vi "Initialization.vi"(8 "error in (no error)":errorcluster, 9 "UI Refs":T1, 10 "user event":T2, 11 "4way Lap in":refnum<class "No Load Drift.lvclass">) -> (0 "error out":errorcluster, 3 "4way Lap out":refnum<class "No Load Drift.lvclass">)   [LabVIEW 2025, in "Flow Grind.lvlib" / "No Load Drift.lvclass"]
uses:
  No Load Drift.lvclass
  Users/Public/Documents/Sandia National Labs/TSS Plugin/CEF.lvlibp/Node/UserEventRef.ctl
  Users/Public/Documents/Sandia National Labs/TSS Plugin/Tests/XY Plotter.lvlibp/XY  Plotter/XY Plotter.lvclass
  Users/Public/Documents/Sandia National Labs/TSS Plugin/CEF.lvlibp/Node/CEF_Node.lvclass
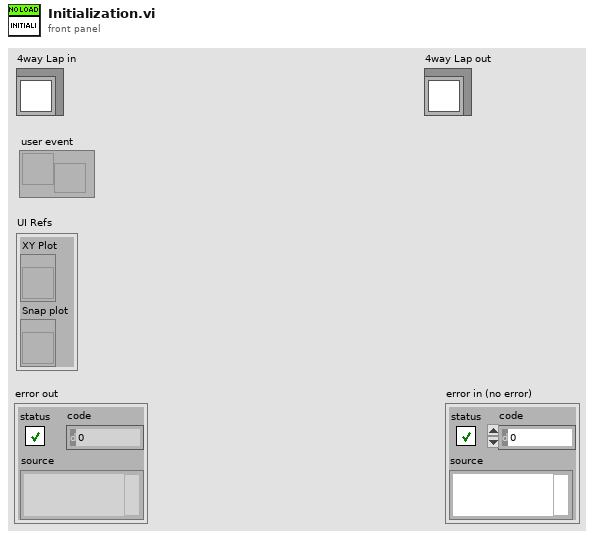
[diagram p1: front panel]
types:
  T1 = cluster{"XY Plot":refnum<vi>, "Snap plot":refnum<vi>}
  T2 = typedef "CEF.lvlibp/CEF_Node.lvclass/UserEventRef.ctl" = refnum<user-event>
  T3 = cluster{"Name":string, "Color":u32, "Style":u8, "Point Style":u8, "Name Visible":bool, "Allow Drag":bool, "Annotation Mode":u32, "Plot":i32, "Index":i32, "Position":cluster{"X":dbl, "Y":dbl}, "X Scale":u32, "Y Scale":u32, "Show Arrow":bool, "Lock Name":bool, "Plot Area":i32, "Label Offset":cluster{"X":dbl, "Y":dbl}}
  T4 = cluster{"Name":string, "Color":u32, "Style":u8, "Point Style":u8, "Name Visible":bool, "Allow Drag":bool, "Annotation Mode":u32, "Plot":i32, "Index":i32, "Position":cluster{"X":dbl, "Y":dbl}, "X Scale":u32, "Y Scale":u32, "Show Arrow":bool, "Lock Name":bool, "Plot Area":i32, "Label Offset":cluster{"X":dbl, "Y":dbl}}[]
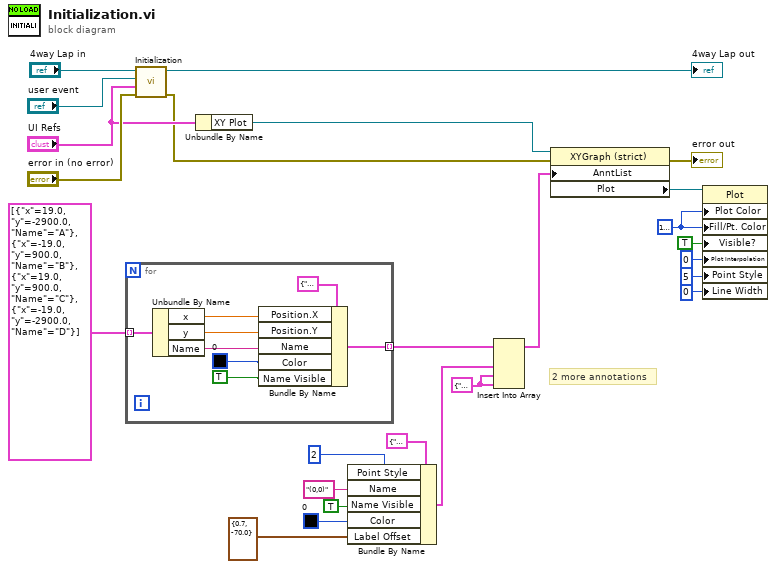
[diagram p0: block diagram]
diagram:
  w8 = T3 {"Name"="", "Color"=0, "Style"=0, "Point Style"=0, "Name Visible"=FALSE, "Allow Drag"=FALSE, "Annotation Mode"=0, "Plot"=0, "Index"=0, "Position"={"X"=0.0, "Y"=0.0}, "X Scale"=0, "Y Scale"=0, "Show Arrow"=FALSE, "Lock Name"=FALSE, "Plot Area"=0, "Label Offset"={"X"=0.0, "Y"=0.0}} ("new element/subarray")
  w17 = u32 16777224 ("Plot Color")
  # "2 more annotations"
  n1 = for {
    tunnel: cluster{"x":dbl, "y":dbl, "Name":string}[] [{"x"=19.0, "y"=-2900.0, "Name"="A"}, {"x"=-19.0, "y"=900.0, "Name"="B"}, {"x"=19.0, "y"=900.0, "Name"="C"}, {"x"=-19.0, "y"=-2900.0, "Name"="D"}] -> [w29] mode=indexing
    tunnel: [w30] -> w12 mode=indexing
    n2 = Unbundle By Name(w29) -> ("x"=w27:dbl, "y"=w26:dbl, "Name"=w28:string)
    n3 = Bundle By Name(cluster=T3 {"Name"="", "Color"=0, "Style"=0, "Point Style"=0, "Name Visible"=FALSE, "Allow Drag"=FALSE, "Annotation Mode"=0, "Plot"=0, "Index"=0, "Position"={"X"=0.0, "Y"=0.0}, "X Scale"=0, "Y Scale"=0, "Show Arrow"=FALSE, "Lock Name"=FALSE, "Plot Area"=0, "Label Offset"={"X"=0.0, "Y"=0.0}}, "Position.X"=w27, "Position.Y"=w26, "Name"=w28, "Color"=u32 0, "Name Visible"=TRUE) -> (w30:T3)
  }
  n4 = call-parent "Initialization.vi"("error in"="error in (no error)", "UI Refs"="UI Refs", "user event"="user event", "XY Plotter"="4way Lap in") -> ("error out"=w14:errorcluster, "XY Plotter out"=→"4way Lap out":refnum<class "No Load Drift.lvclass">)  [unwired: 6 in]
  n5 = Unbundle By Name("UI Refs") -> ("XY Plot"=w10:refnum<vi>)
  n6 = Bundle By Name(cluster=T3 {"Name"="", "Color"=0, "Style"=0, "Point Style"=0, "Name Visible"=FALSE, "Allow Drag"=FALSE, "Annotation Mode"=0, "Plot"=0, "Index"=0, "Position"={"X"=0.0, "Y"=0.0}, "X Scale"=0, "Y Scale"=0, "Show Arrow"=FALSE, "Lock Name"=FALSE, "Plot Area"=0, "Label Offset"={"X"=0.0, "Y"=0.0}} ("new element/subarray"), "Point Style"=u8 2, "Name"="(0,0)", "Name Visible"=TRUE, "Color"=u32 0, "Label Offset"=cluster{"X":dbl, "Y":dbl} {"X"=0.7, "Y"=-70.0}) -> (w1:T3)
  n7 = Insert Into Array(array=w12, new element #1=w1, new element #2=w8, new element #3=w8) -> (w11:T4)  [unwired: 1 in]
  n8 = property class="XYGraph (strict)"(reference=w10, error in=w14, "AnntList"=w11) -> (error out=→"error out":errorcluster, "Plot"=w9:refnum<vi>)  [unwired: 1 out]
  n9 = property class="Plot"(reference=w9, "Plot Color"=w17, "Fill/Pt. Color"=w17, "Visible?"=TRUE ("Visible"), "Plot Interpolation"=u8 0, "Point Style"=u8 5, "Line Width"=u8 0) -> ()  [unwired: 1 in, 2 out]
